vi "XNET.Settings.vi"(6 "Action":enum8{"Get", "Set"}(ring), 8 "error in (no error)":errorcluster, 10 "XNET Settings":T1={"Database"="", "Cluster"="", "Port"="", "Baud rate [Bd]"=500000, "Termination"=1, "CAN I/O Mode"=0, "FD Baud rate [Bd]"=500000, "Priority"=100, "Use Legacy"=FALSE, "FD ISO Mode"=0, "Default Max Counter Value"=0.0, "Default Protect Type"=enum."Arb ID + Bytes Checksum with Inversion", "Include All Channels"=FALSE} {"FD ISO Mode" items=["ISO", "Non ISO", "ISO Legacy"]; "CAN I/O Mode" items=["CAN 2.0", "CAN FD", "CAN FD+BRS"]; "Termination" items=["Off", "On"]}, 11 "Parent Ref in":T3 format="%.0x") -> (0 "error out":errorcluster, 2 "XNET Settings":T1={"Database"="", "Cluster"="", "Port"="", "Baud rate [Bd]"=500000, "Termination"=1, "CAN I/O Mode"=0, "FD Baud rate [Bd]"=500000, "Priority"=100, "Use Legacy"=FALSE, "FD ISO Mode"=0, "Default Max Counter Value"=0.0, "Default Protect Type"=enum."Arb ID + Bytes Checksum with Inversion", "Include All Channels"=FALSE} {"FD ISO Mode" items=["ISO", "Non ISO", "ISO Legacy"]; "CAN I/O Mode" items=["CAN 2.0", "CAN FD", "CAN FD+BRS"]; "Termination" items=["Off", "On"]}, 3 "Item Ref out":T3 format="%.0x")   [LabVIEW 2025, in "Protection and Counter Addon System Explorer.lvlib"]
uses:
  Protection and Counter Addon System Explorer.lvlib
  Addon Shared/Types/XNET Settings.ctl
  SubModules/Frame-Protection-Support/Source/Shared/Types/Protection Type.ctl
  <vilib>/NI VeriStand/Custom Device API/Custom Device Item Ref.ctl
  Addon Shared/SubVIs/GUID Lookup.vi
  <vilib>/NI/NI VeriStand Advanced SysDef API/_SubVIs/SysDef.Property.Set.String.vi
  <vilib>/NI/NI VeriStand Advanced SysDef API/_SubVIs/SysDef.Property.Set.U64.vi
  <vilib>/NI/NI VeriStand Advanced SysDef API/_SubVIs/SysDef.Property.Set.U32.vi
  <vilib>/NI/NI VeriStand Advanced SysDef API/_SubVIs/SysDef.Property.Set.I32.vi
  <vilib>/NI/NI VeriStand Advanced SysDef API/_SubVIs/SysDef.Property.Set.Boolean.vi
  <vilib>/NI/NI VeriStand Advanced SysDef API/_SubVIs/SysDef.Property.Set.DBL.vi
  <vilib>/NI/NI VeriStand Advanced SysDef API/SysDef API/Advanced System Definition.lvlib
  Addon Shared/Protection and Counter Addon Shared.lvlib
  <vilib>/NI/NI VeriStand Advanced SysDef API/_SubVIs/SysDef.Property.Get.String.vi
  <vilib>/NI/NI VeriStand Advanced SysDef API/_SubVIs/SysDef.Property.Get.U64.vi
  <vilib>/NI/NI VeriStand Advanced SysDef API/_SubVIs/SysDef.Property.Get.U32.vi
  <vilib>/NI/NI VeriStand Advanced SysDef API/_SubVIs/SysDef.Property.Get.I32.vi
  <vilib>/NI/NI VeriStand Advanced SysDef API/_SubVIs/SysDef.Property.Get.Boolean.vi
  <vilib>/NI/NI VeriStand Advanced SysDef API/_SubVIs/SysDef.Property.Get.DBL.vi
  <vilib>/NI VeriStand/Custom Device API/Custom Device API.lvlib
  SubModules/Frame-Protection-Support/Source/Shared/Protection and Counter Support Shared.lvlib
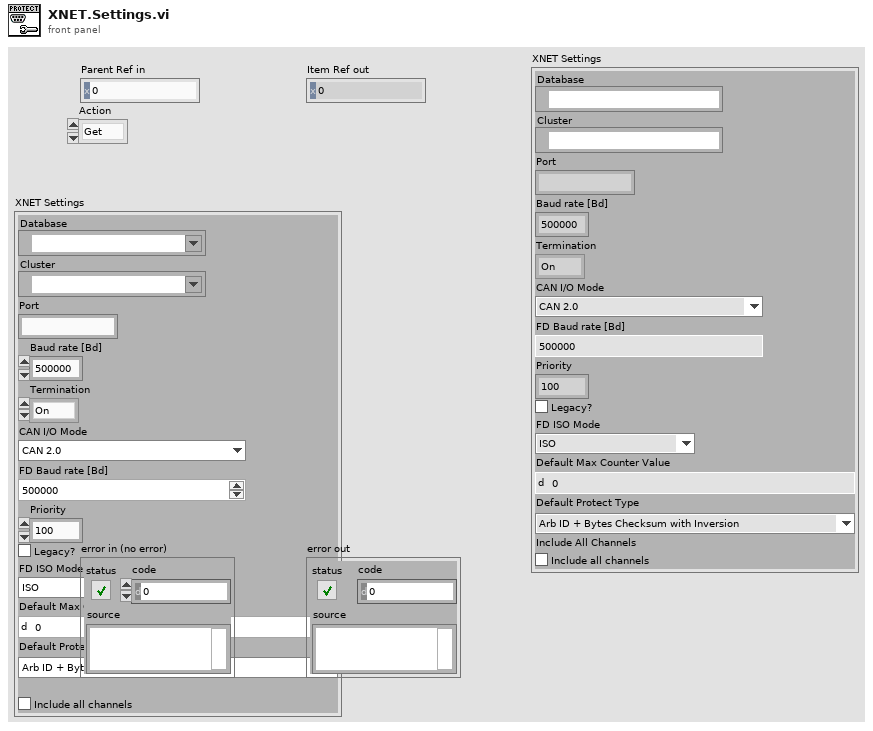
[diagram p1: front panel]
types:
  T1 = typedef "Protection and Counter Addon Shared.lvlib/XNET Settings.ctl" = cluster{"Database":refnum<k21>, "Cluster":refnum<k21>, "Port":string, "Baud rate [Bd]":u64, "Termination":u32, "CAN I/O Mode":u32, "FD Baud rate [Bd]":u64, "Priority":i32, "Use Legacy":bool, "FD ISO Mode":u32, "Default Max Counter Value":dbl, "Default Protect Type":T2, "Include All Channels":bool}
  T2 = typedef "Protection and Counter Support Shared.lvlib/Protection Type.ctl" = enum16{"Arb ID + Bytes Checksum with Inversion", "Arb ID + Bytes CRC with Inversion", "Reversed Raw Signal Checksum with Inversion", "Concatenated Two's Compliment"}
  T3 = typedef "Custom Device API.lvlib/Custom Device Item Ref.ctl" = u64
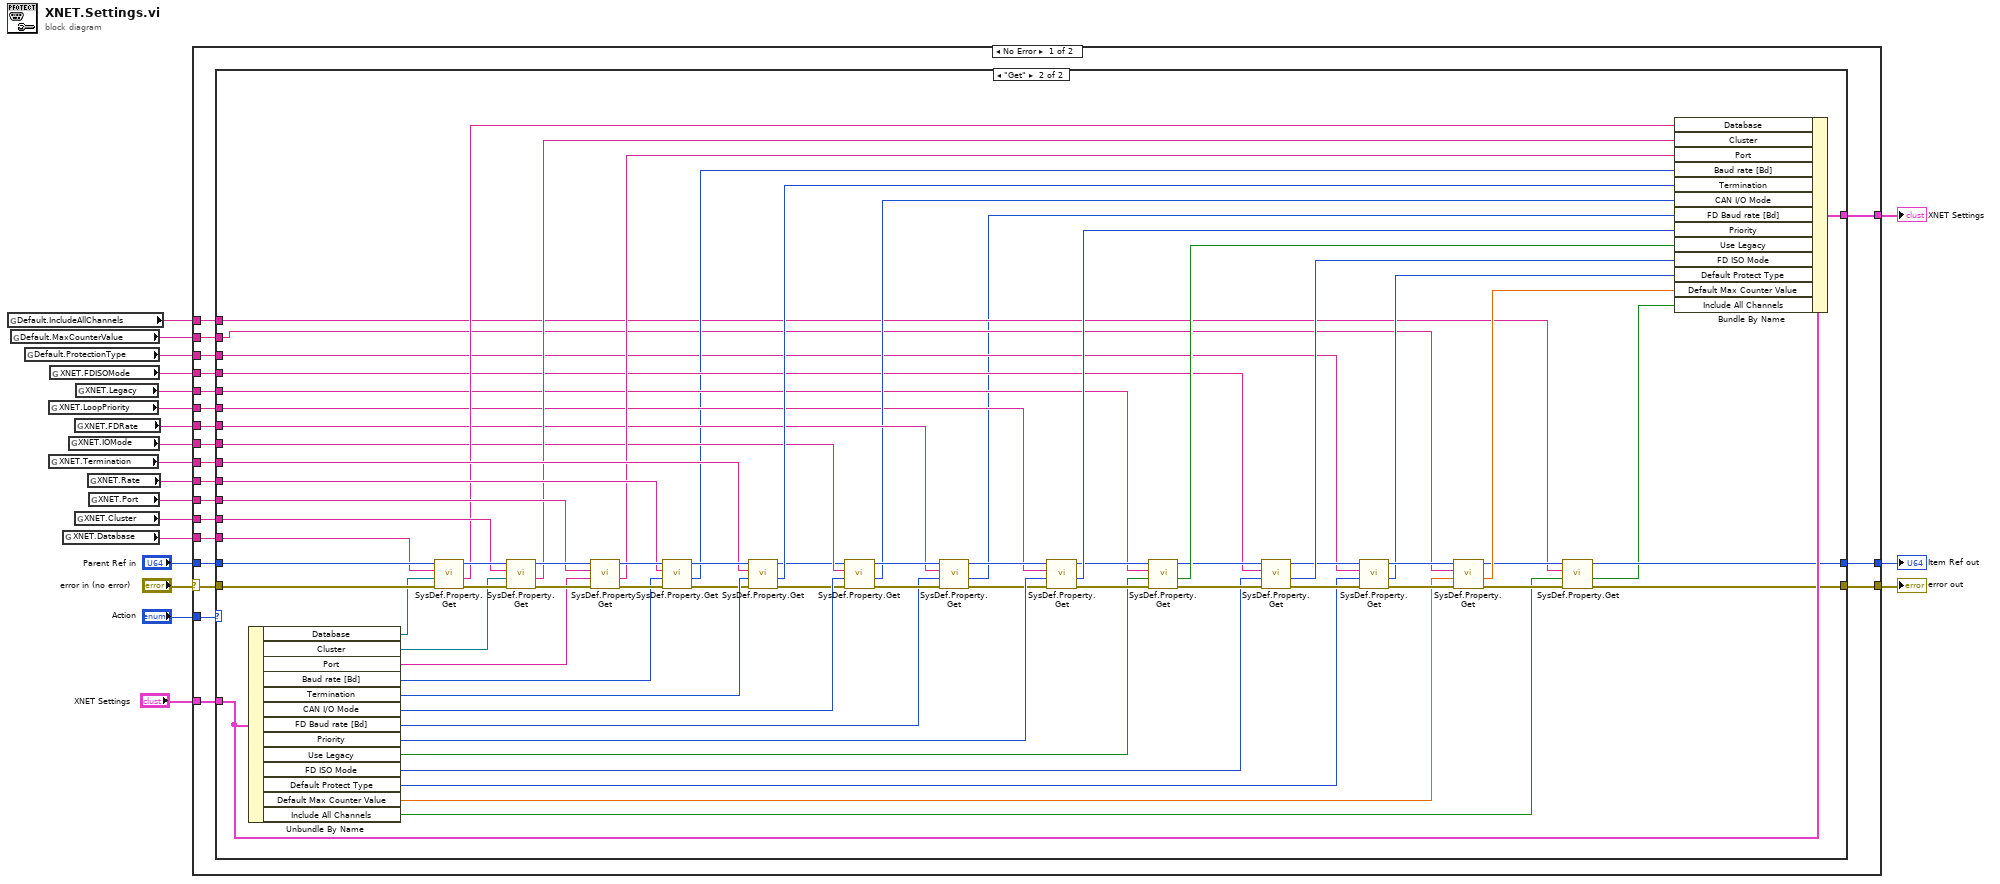
[diagram p0: block diagram]
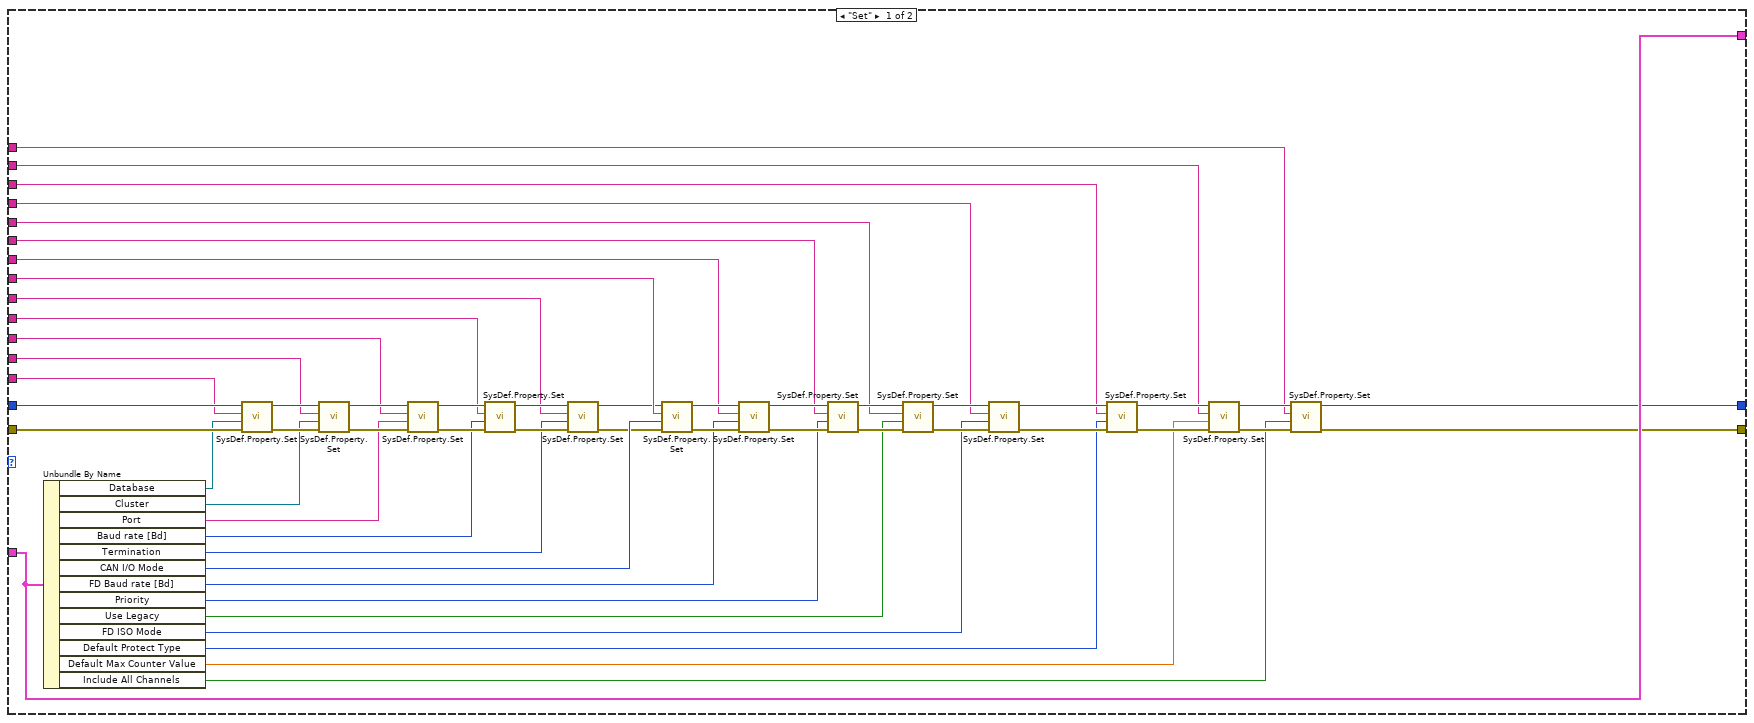
[diagram p2: hidden frame]
diagram:
  n1 = global read "GUID Lookup.vi" "Default.IncludeAllChannels"() -> (w1:string)
  n2 = global read "GUID Lookup.vi" "Default.MaxCounterValue"() -> (w3:string)
  n3 = global read "GUID Lookup.vi" "Default.ProtectionType"() -> (w2:string)
  n4 = global read "GUID Lookup.vi" "XNET.LoopPriority"() -> (w6:string)
  n5 = global read "GUID Lookup.vi" "XNET.Termination"() -> (w9:string)
  n6 = global read "GUID Lookup.vi" "XNET.FDISOMode"() -> (w4:string)
  n7 = global read "GUID Lookup.vi" "XNET.Database"() -> (w13:string)
  n8 = global read "GUID Lookup.vi" "XNET.IOMode"() -> (w8:string)
  n9 = global read "GUID Lookup.vi" "XNET.FDRate"() -> (w7:string)
  n10 = global read "GUID Lookup.vi" "XNET.Cluster"() -> (w12:string)
  n11 = global read "GUID Lookup.vi" "XNET.Legacy"() -> (w5:string)
  n12 = global read "GUID Lookup.vi" "XNET.Rate"() -> (w10:string)
  n13 = global read "GUID Lookup.vi" "XNET.Port"() -> (w11:string)
  n14 = case shown="No Error" "error in (no error)" {
    selector: "error in (no error)" -> [w31 w167]
    tunnel: "Parent Ref in" -> [w40 w166]
    tunnel: w13 -> [w39 _]
    tunnel: "XNET Settings" -> [w38 w165]
    tunnel: [w37 w167] -> w18
    tunnel: [w36 w166] -> w17
    tunnel: w12 -> [w35 _]
    tunnel: w11 -> [w34 _]
    tunnel: w9 -> [w33 _]
    tunnel: w10 -> [w32 _]
    tunnel: "Action" -> [w30 _]
    tunnel: [w29 w165] -> w14
    tunnel: w8 -> [w28 _]
    tunnel: w7 -> [w27 _]
    tunnel: w6 -> [w26 _]
    tunnel: w5 -> [w25 _]
    tunnel: w4 -> [w24 _]
    tunnel: w3 -> [w23 _]
    tunnel: w2 -> [w22 _]
    tunnel: w1 -> [w21 _]
    frame No Error {
      n15 = case shown="\"Get\"" w30 {
        tunnel: w40 -> [w95 w164]
        tunnel: w39 -> [w94 w163]
        tunnel: w38 -> [w76 w146]
        tunnel: [w41 w102] -> w37
        tunnel: [w42 w101] -> w36
        tunnel: w35 -> [w81 w155]
        tunnel: w34 -> [w80 w154]
        tunnel: w33 -> [w79 w153]
        tunnel: w32 -> [w78 w152]
        tunnel: w31 -> [w77 w151]
        tunnel: [w76 w141] -> w29
        tunnel: w28 -> [w72 w137]
        tunnel: w27 -> [w71 w136]
        tunnel: w26 -> [w63 w129]
        tunnel: w25 -> [w60 w123]
        tunnel: w24 -> [w56 w119]
        tunnel: w23 -> [w48 w108]
        tunnel: w22 -> [w47 w107]
        tunnel: w21 -> [w44 w100]
        frame "Set" {
          n16 = Unbundle By Name(w76) -> ("Database"=w75:refnum<k21>, "Cluster"=w85:refnum<k21>, "Port"=w84:string, "Baud rate [Bd]"=w83:u64, "Termination"=w82:u32, "CAN I/O Mode"=w70:u32, "FD Baud rate [Bd]"=w69:u64, "Priority"=w64:i32, "Use Legacy"=w59:bool, "FD ISO Mode"=w55:u32, "Default Protect Type"=w50:T2, "Default Max Counter Value"=w49:dbl, "Include All Channels"=w43:bool)
          n17 = call-poly <vilib>:"SysDef.Property.Set.vi"("error in (no error)"=w77, "Value"=w75, "Property Name"=w94, "nodeID"=w95) -> ("error out"=w91:errorcluster, "nodeID out"=w90:u64)  [unwired: 6 in]
          n18 = call-poly <vilib>:"SysDef.Property.Set.vi"("error in (no error)"=w91, "Value"=w85, "Property Name"=w81, "nodeID"=w90) -> ("error out"=w92:errorcluster, "nodeID out"=w93:u64)  [unwired: 6 in]
          n19 = call-poly <vilib>:"SysDef.Property.Set.vi"("error in (no error)"=w92, "Value"=w84, "Property Name"=w80, "nodeID"=w93) -> ("error out"=w87:errorcluster, "nodeID out"=w86:u64)  [unwired: 6 in]
          n20 = call-poly <vilib>:"SysDef.Property.Set.vi"("error in (no error)"=w87, "Value"=w83, "Property Name"=w78, "nodeID"=w86) -> ("error out"=w88:errorcluster, "nodeID out"=w89:u64)  [unwired: 6 in]
          n21 = call-poly <vilib>:"SysDef.Property.Set.vi"("error in (no error)"=w88, "Value"=w82, "Property Name"=w79, "nodeID"=w89) -> ("error out"=w68:errorcluster, "nodeID out"=w67:u64)  [unwired: 6 in]
          n22 = call-poly <vilib>:"SysDef.Property.Set.vi"("error in (no error)"=w68, "Value"=w70, "Property Name"=w72, "nodeID"=w67) -> ("error out"=w74:errorcluster, "nodeID out"=w73:u64)  [unwired: 6 in]
          n23 = call-poly <vilib>:"SysDef.Property.Set.vi"("error in (no error)"=w74, "Value"=w69, "Property Name"=w71, "nodeID"=w73) -> ("error out"=w66:errorcluster, "nodeID out"=w65:u64)  [unwired: 6 in]
          n24 = call-poly <vilib>:"SysDef.Property.Set.vi"("error in (no error)"=w66, "Value"=w64, "Property Name"=w63, "nodeID"=w65) -> ("error out"=w62:errorcluster, "nodeID out"=w61:u64)  [unwired: 6 in]
          n25 = call-poly <vilib>:"SysDef.Property.Set.vi"("error in (no error)"=w62, "Value"=w59, "Property Name"=w60, "nodeID"=w61) -> ("error out"=w58:errorcluster, "nodeID out"=w57:u64)  [unwired: 6 in]
          n26 = call-poly <vilib>:"SysDef.Property.Set.vi"("error in (no error)"=w58, "Value"=w55, "Property Name"=w56, "nodeID"=w57) -> ("error out"=w54:errorcluster, "nodeID out"=w53:u64)  [unwired: 6 in]
          n27 = call-poly <vilib>:"SysDef.Property.Set.vi"("error in (no error)"=w54, "Value"=w50, "Property Name"=w47, "nodeID"=w53) -> ("error out"=w52:errorcluster, "nodeID out"=w51:u64)  [unwired: 6 in]
          n28 = call-poly <vilib>:"SysDef.Property.Set.vi"("error in (no error)"=w52, "Value"=w49, "Property Name"=w48, "nodeID"=w51) -> ("error out"=w46:errorcluster, "nodeID out"=w45:u64)  [unwired: 6 in]
          n29 = call-poly <vilib>:"SysDef.Property.Set.vi"("error in (no error)"=w46, "Value"=w43, "Property Name"=w44, "nodeID"=w45) -> ("error out"=w41:errorcluster, "nodeID out"=w42:u64)  [unwired: 6 in]
        }
        frame "Get" {
          n30 = Unbundle By Name(w146) -> ("Database"=w150:refnum<k21>, "Cluster"=w149:refnum<k21>, "Port"=w148:string, "Baud rate [Bd]"=w131:u64, "Termination"=w147:u32, "CAN I/O Mode"=w138:u32, "FD Baud rate [Bd]"=w134:u64, "Priority"=w128:i32, "Use Legacy"=w122:bool, "FD ISO Mode"=w118:u32, "Default Protect Type"=w105:T2, "Default Max Counter Value"=w106:dbl, "Include All Channels"=w99:bool)
          n31 = call-poly <vilib>:"SysDef.Property.Get.vi"("error in (no error)"=w151, "Value"=w150, "Property Name"=w163, "nodeID"=w164) -> ("error out"=w160:errorcluster, "Value out"=w145:string, "nodeID out"=w159:u64)  [unwired: 4 in, 1 out]
          n32 = call-poly <vilib>:"SysDef.Property.Get.vi"("error in (no error)"=w160, "Value"=w149, "Property Name"=w155, "nodeID"=w159) -> ("error out"=w161:errorcluster, "Value out"=w144:string, "nodeID out"=w162:u64)  [unwired: 4 in, 1 out]
          n33 = call-poly <vilib>:"SysDef.Property.Get.vi"("error in (no error)"=w161, "Value"=w148, "Property Name"=w154, "nodeID"=w162) -> ("error out"=w157:errorcluster, "Value out"=w143:string, "nodeID out"=w156:u64)  [unwired: 4 in, 1 out]
          n34 = call-poly <vilib>:"SysDef.Property.Get.vi"("error in (no error)"=w157, "Value"=w131, "Property Name"=w152, "nodeID"=w156) -> ("error out"=w116:errorcluster, "Value out"=w115:u64, "nodeID out"=w158:u64)  [unwired: 4 in, 1 out]
          n35 = call-poly <vilib>:"SysDef.Property.Get.vi"("error in (no error)"=w116, "Value"=w147, "Property Name"=w153, "nodeID"=w158) -> ("error out"=w132:errorcluster, "Value out"=w142:u32, "nodeID out"=w133:u64)  [unwired: 4 in, 1 out]
          n36 = call-poly <vilib>:"SysDef.Property.Get.vi"("error in (no error)"=w132, "Value"=w138, "Property Name"=w137, "nodeID"=w133) -> ("error out"=w140:errorcluster, "Value out"=w135:u32, "nodeID out"=w139:u64)  [unwired: 4 in, 1 out]
          n37 = call-poly <vilib>:"SysDef.Property.Get.vi"("error in (no error)"=w140, "Value"=w134, "Property Name"=w136, "nodeID"=w139) -> ("error out"=w97:errorcluster, "Value out"=w96:u64, "nodeID out"=w130:u64)  [unwired: 4 in, 1 out]
          n38 = call-poly <vilib>:"SysDef.Property.Get.vi"("error in (no error)"=w97, "Value"=w128, "Property Name"=w129, "nodeID"=w130) -> ("error out"=w126:errorcluster, "Value out"=w127:i32, "nodeID out"=w125:u64)  [unwired: 4 in, 1 out]
          n39 = call-poly <vilib>:"SysDef.Property.Get.vi"("error in (no error)"=w126, "Value"=w122, "Property Name"=w123, "nodeID"=w125) -> ("error out"=w121:errorcluster, "Value out"=w124:bool, "nodeID out"=w120:u64)  [unwired: 4 in, 1 out]
          n40 = call-poly <vilib>:"SysDef.Property.Get.vi"("error in (no error)"=w121, "Value"=w118, "Property Name"=w119, "nodeID"=w120) -> ("error out"=w113:errorcluster, "Value out"=w117:u32, "nodeID out"=w114:u64)  [unwired: 4 in, 1 out]
          n41 = call-poly <vilib>:"SysDef.Property.Get.vi"("error in (no error)"=w113, "Value"=w105, "Property Name"=w107, "nodeID"=w114) -> ("error out"=w112:errorcluster, "Value out"=w109:u32, "nodeID out"=w111:u64)  [unwired: 4 in, 1 out]
          n42 = call-poly <vilib>:"SysDef.Property.Get.vi"("error in (no error)"=w112, "Value"=w106, "Property Name"=w108, "nodeID"=w111) -> ("error out"=w103:errorcluster, "Value out"=w110:dbl, "nodeID out"=w104:u64)  [unwired: 4 in, 1 out]
          n43 = call-poly <vilib>:"SysDef.Property.Get.vi"("error in (no error)"=w103, "Value"=w99, "Property Name"=w100, "nodeID"=w104) -> ("error out"=w102:errorcluster, "Value out"=w98:bool, "nodeID out"=w101:u64)  [unwired: 4 in, 1 out]
          n44 = Bundle By Name(cluster=w146, "Database"=w145, "Cluster"=w144, "Port"=w143, "Baud rate [Bd]"=w115, "Termination"=w142, "CAN I/O Mode"=w135, "FD Baud rate [Bd]"=w96, "Priority"=w127, "Use Legacy"=w124, "FD ISO Mode"=w117, "Default Protect Type"=w109, "Default Max Counter Value"=w110, "Include All Channels"=w98) -> (w141:T1)
        }
      }
    }
    frame Error {
    }
  }
  "Item Ref out" <- w17
  "error out" <- w18
  "XNET Settings" <- w14
